vi "ExecutingCalibration.vi"(8 "error in (no error)":errorcluster, 10 "calibration_id":i32, 11 "ByteQXAPIBase in":refnum<class "ByteQXAPIBase.lvclass">) -> (0 "error out":errorcluster, 2 "calibration data":T1 {"controls"."umidita" format="%.1g"; "controls"."temperatura_c" format="%.1g"; "controls"."incertezza" format="%.1g"; "controls"."deviazione_standard" format="%.1g"; "controls"."mpe_min" format="%.1g"; "controls"."mpe_max" format="%.1g"; "controls"."riferimento_obiettivo" format="%.1g"}, 3 "ByteQXAPIBase out":refnum<class "ByteQXAPIBase.lvclass">)   [LabVIEW 2019, in "ByteQXWebAPI.lvlib" / "ByteQXAPIBase.lvclass"]
doc: "Obtain calibration measurements for the specified calibration Id"
uses:
  ByteQXAPIBase.lvclass
  CalibMeasure.ctl
  <vilib>/Bytelabs/ByteREST/ByteRESTClass/ByteRESTBase/HTTP/Status_Code.ctl
  Private/module.ctl
  ByteQXAPIBase.lvclass/ByteQXAPIBase.ctl
  <vilib>/Utility/error.llb/Error Cluster From Error Code.vi
  <vilib>/ErrorRing/Error Ring.xnode
  <vilib>/Bytelabs/ByteREST/ByteRESTClass/ByteRESTBase/RESTBase.lvclass
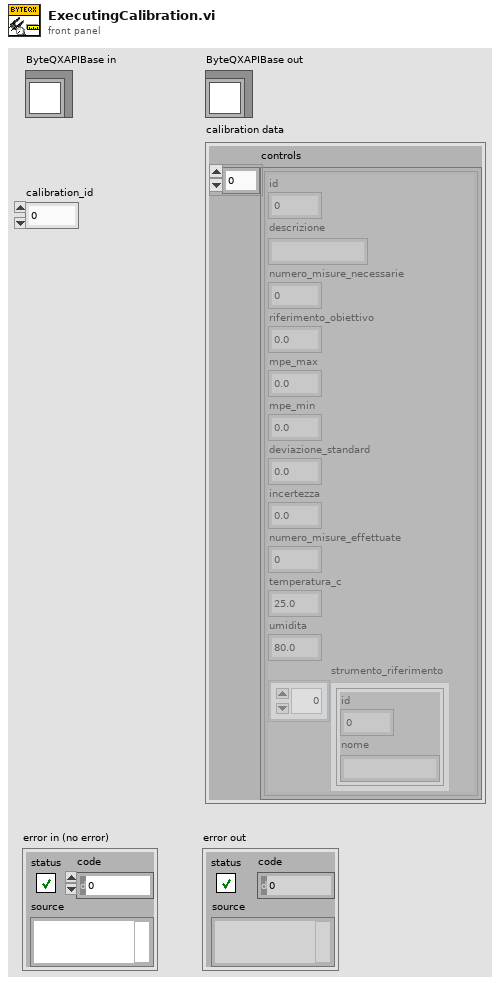
[diagram p1: front panel]
types:
  T1 = typedef "ByteQXWebAPI.lvlib/ByteQXAPIBase.lvclass/CalibMeasure.ctl" = cluster{"controls":cluster{"id":u16, "descrizione":string, "numero_misure_necessarie":u16, "riferimento_obiettivo":dbl, "mpe_max":dbl, "mpe_min":dbl, "deviazione_standard":dbl, "incertezza":dbl, "numero_misure_effettuate":u32, "temperatura_c":dbl, "umidita":dbl, "strumento_riferimento":cluster{"id":u16, "nome":string}[]}[]}
  T2 = typedef "ByteQXWebAPI.lvlib/ByteQXAPIBase.lvclass/module.ctl" = enum16{"gs", "tms", "data"}
  T3 = typedef "ByteREST.lvlib/RESTBase.lvclass/Status_Code.ctl" = u16
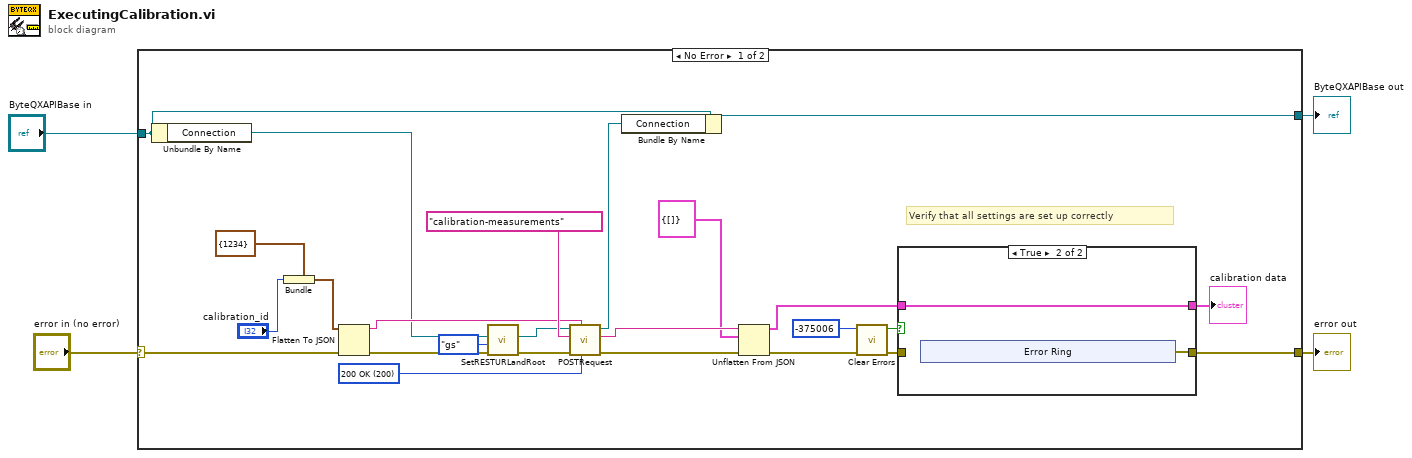
[diagram p0: block diagram]
diagram:
  n1 = case shown="No Error" "error in (no error)" {
    selector: "error in (no error)" -> [w25 w40]
    tunnel: [w13 w40] -> w3
    tunnel: [w28 w39] -> w1
    tunnel: "ByteQXAPIBase in" -> [w29 w39]
    frame No Error {
      w22 = T3 200 items=["200 OK"=200, "201 Created"=201, "400 Bad Request"=400, "401 Unauthorized"=401, "403 Forbidden"=403, "404 Not Found"=404, "405 Method Not Allowed"=405, "406 Not Acceptable"=406, "500 Internal Server Error"=500] ("expected response")
      # "Verify that all settings are set up correctly"
      n2 = Unbundle By Name(w29) -> ("Connection"=w7:refnum<class "RESTBase.lvclass">)
      n3 = Bundle(cluster=cluster{"calibration_id":i32} {"calibration_id"=1234}, "calibration_id"="calibration_id") -> (w17:cluster{"calibration_id":i32})
      n4 = Flatten To JSON(anything=w17, error in (no error)=w25) -> (JSON string=w21:string, 11:w9:errorcluster)  [unwired: 1 in]
      n5 = call "SetRESTURLandRoot.vi"("error in (no error)"=w9, "module"=module."gs", "ByteREST in"=w7) -> ("error out"=w8:errorcluster, "ByteREST out"=w6:refnum<class "RESTBase.lvclass">)  [unwired: 7 in]
      n6 = call-dynamic "POSTRequest.vi"("expected response"=w22, "Body in"=w21, "error in (no error)"=w8, "Request"="calibration-measurements", "ByteRESTBase in"=w6) -> ("error out"=w23:errorcluster, "Body"=w24:string, "ByteRESTBase out"=w27:refnum<class "RESTBase.lvclass">)  [unwired: 3 in, 1 out]
      n7 = Bundle By Name(cluster=w29, "Connection"=w27) -> (w28:refnum<class "ByteQXAPIBase.lvclass">)
      n8 = Unflatten From JSON(JSON string=w24, type and defaults=T1 {"controls"=[]} ("Cluster 2"), error in (no error)=w23) -> (value=w11:T1, error out=w15:errorcluster)  [unwired: 4 in]
      n9 = call <vilib>:"Clear Errors.vi"("error in (no error)"=w15, "specific error code to clear (0: all)"=-375006 ("error code (no error:0)")) -> ("error out"=w14:errorcluster, "specific error cleared?"=w12:bool)  [unwired: 4 in]
      n10 = case shown="True" w12 {
        tunnel: w14 -> [w31 _]
        tunnel: [w31 w32] -> w13
        tunnel: w11 -> [w30 w33]
        tunnel: [w30 w33] -> w10
        frame False {
        }
        frame True {
          n11 = xnode "Error Ring"() -> ("error out"=w32:errorcluster)
        }
      }
      "calibration data" <- w10
    }
    frame Error {
    }
  }
  "error out" <- w3
  "ByteQXAPIBase out" <- w1
